vi "[ce] ODE Solver - Preparation.vi"(4 "method":enum16{"Runge Kutta", "Euler"}(ring), 6 "equation parameters":T1(array[cluster]) {"x0" format="%.2f"}, 8 "error in":errorcluster, 9 "h value":dbl format="%.3f", 10 "time value":dbl format="%.2f", 11 "time":string="t") -> (0 "error out":errorcluster, 2 "expression":string, 3 "VC Handle":T2=-1, 5 "var names":string[](array[string]), 7 "X0":dbl[](array[numeric]) format="%.2f")   [LabVIEW 2021]
doc: "::: CalcExpress Toolkit :::\nCopyright (c) 2000-2026 Konstantin Shifershteyn. All rights reserved."
uses:
  cetypes.llb/VarMan Variable Context Handle.ctl
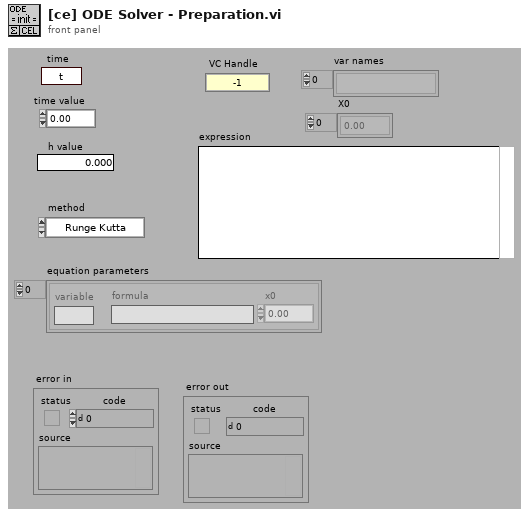
[diagram p1: front panel]
types:
  T1 = cluster{"variable":string, "formula":string, "x0":dbl}[]
  T2 = typedef "VarMan Variable Context Handle.ctl" = i32
  T3 = cluster{"var":string, "var_tmp":string, "var_k1":string, "var_k2":string, "var_k3":string, "var_k4":string}[]
  T4 = cluster{"time":string, "time 0":string, "iteration":string, "step":string, "half step":string}
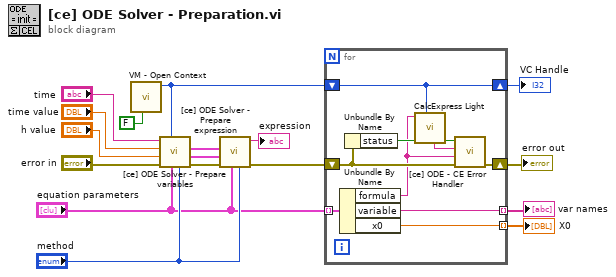
[diagram p0: block diagram]
diagram:
  n1 = call "VM - Open Context.vi"("close loose contexts (F)"=FALSE ("close loose contexts (T)")) -> ("VC Handle out"=w13:T2)  [unwired: 8 in, 2 out]
  n2 = call "[ce] ODE Solver - Prepare variables.vi"("method"="method", "equation parameters"="equation parameters", "VC Handle"=w13, "error in"="error in", "h value"="h value", "time value"="time value", "time"="time") -> ("error out"=w15:errorcluster, "variable names"=w16:T3, "time names"=w17:T4)  [unwired: 1 in, 1 out]
  n3 = call "[ce] ODE Solver - Prepare expression.vi"("method"="method", "equation parameters"="equation parameters", "error in"=w15, "variable names"=w16, "time names"=w17) -> ("error out"=w14:errorcluster, "expression"=→"expression":string)  [unwired: 5 in]
  n4 = for {
    shift-right: [w27] -> w8
    shift-left: w13 -> [w27]
    shift-right: [w22] -> w7
    shift-left: w14 -> [w24]
    tunnel: "equation parameters" -> [w21] mode=indexing
    tunnel: [w19] -> w3 mode=indexing
    tunnel: [w18] -> w2 mode=indexing
    n5 = Unbundle By Name(w21) -> ("formula"=w20:string, "variable"=w19:string, "x0"=w18:dbl)
    n6 = Unbundle By Name(w24) -> ("status"=w26:bool)
    n7 = call "CalcExpress Light.vi"("VC Handle"=w27, "error in"=w26, "expression"=w20) -> ("error out"=w25:bool, "error description"=w23:string)  [unwired: 5 in, 2 out]
    n8 = call "[ce] ODE - CE Error Handler.vi"("error before"=w24, "formula"=w20, "message"=w23, "error"=w25) -> ("error out"=w22:errorcluster)  [unwired: 5 in]
  }
  "VC Handle" <- w8
  "error out" <- w7
  "var names" <- w3
  "X0" <- w2
